vi "Variable glob Keller.vi"() -> ()   [LabVIEW 2022 SP3]
panel:
  in  "Refnum Keller":refnum<vi>
  in  "Noms KELLER selectionnes":string[](array[string])
  out "Selection KELLER":bool[](array[boolean])=[TRUE]
  in  "Port COM KELLER":refnum<visa-resource-name>="COM11"
  in  "Adresses KELLER":i16[](array[numeric])=[10]
  in  "Noms KELLER":string[](array[string])=["PT160"]
  in  "Donnees KELLER":string[](array[string])
  in  "KELLER":bool=TRUE
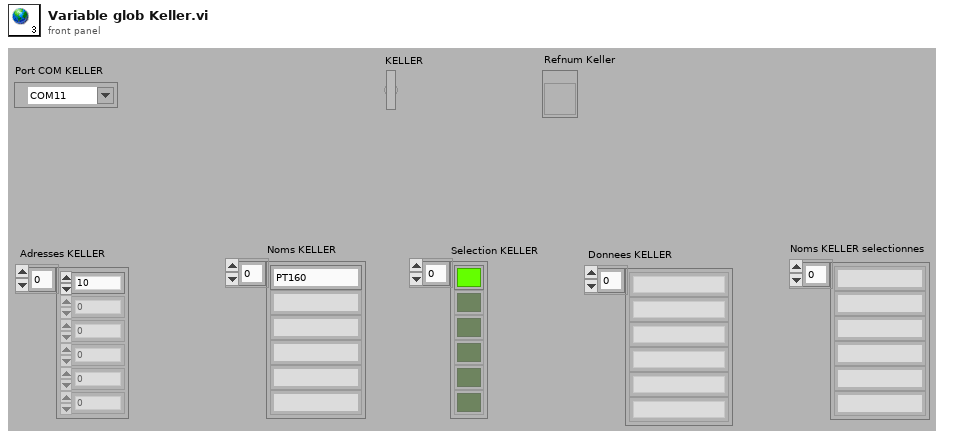
[diagram p1: front panel]
diagram:
